vi "CSM - Run Script.vi"(0 "CSM Scripts":string, 1 "Current Module (\"\" to Generate an ID)":string, 7 "Continue If Error? (F)":bool, 9 "Wait (5000ms)":i32=5000, 11 "error in (no error)":errorcluster, 12 "Response Timeout (-2 Using Global Settings)":i32=-2) -> (4 "Response":string[](array[string]), 10 "Scripts Left":string, 15 "error out":errorcluster)   [LabVIEW 2017, in "Communicable State Machine.lvlib"]
doc: "Executes multiple CSM commands in a single batch, supporting synchronous messages, asynchronous messages, and registrations.\n\n<b>Temporary Variable Support</b>\n\nCSM - Run Script.vi supports an additional supplementary syntax to save return values to specified temporary variables for use in subsequent instructions. Use the `=>` symbol to save the return value to a variable, and variable names are case-insensitive. In subsequent instructions, you can reference the variable using the syntax `${variable name}`.\n\nExample:\n\n```\nAPI: Random -@ csm => var1\nAPI: Random -@ csm => var2\nAPI: echo >> ${var1} -@ csm\nAPI: echo >> ${var2} -@ csm\nAPI: echo >> ${var1},${var2} -@ csm\n```\n\n<b>Additional Command</b>\n\n- Wait: Wait for the specified number of milliseconds, for example `Wait: 1000` means wait 1000 milliseconds.\n\n```\nAPI: Do Something -@ csm\nWait: 1000 // Wait 1000 milliseconds, then continue to the next instruction\nAPI: Do Something Else -@ csm\n```\n\n> [!WARNING]\n> <b>Temporary Variable Support</b> and <b>Additional Command</b> are not natively supported by CSM, but are parsed and processed by CSM - Run Script.vi. Therefore, temporary variables can only be used within the same script execution and cannot be saved or passed across scripts. Wait is also not part of the CSM instructions and cannot use this syntax elsewhere.\n\n\n> [!NOTE] <b>CSM Message Target Module Description</b>\n>\n> In Normal Mode, the target module for a CSM message is the specified module name.\n> System-level modules start with a `.` in their name. The target module for a CSM message includes the `.` in the name. For example, if the requested module name is `.System`, the target module for the CSM message is `.System`.\n> In Worker Mode, the target module for a CSM message can only be the overall module name, not the node name. For example, if the requested module name is `Worker#`, the target module for the CSM message is `Worker`.\n> In Chain of Responsibility Mode, the target module for a CSM message can only be the overall module name, not the node name. For example, if the requested module name is `Chain$1`, the target module for the CSM message is `Chain`.\n\n\n-- <b>Controls</b> --\n- <b>Current Module (\"\" to Generate an ID)</b>: Name of the current module. If empty, a temporary ID is generated for debugging purposes to identify the location.\n- <b>CSM Scripts</b>: CSM commands to execute.\n- <b>Continue If Error? (F)</b>: Whether to continue execution if an error occurs. The default is FALSE, which specifies to not continue.\n- <b>Wait (5000 ms)</b>: Timeout duration for waiting module to be alive. The default is 5000 ms.\n- <b>Response Timeout (-2 Using Global Settings)</b>: Timeout for synchronous calls. The default is -2, which uses the global setting. You can set the global timeout using the CSM - Set TMO of Sync-Reply VI.\n\n-- <b>Indicators</b> --\n- <b>Response</b>: Returned results from executing the script. Only synchronous messages carry returns. The corresponding column for other commands will be an empty string.\n- <b>Scripts Left</b>: Remaining unexecuted scripts."
uses:
  Communicable State Machine.lvlib
  CSM - Broadcast Message Type.ctl
  _Shared/CSM Shared.lvlib
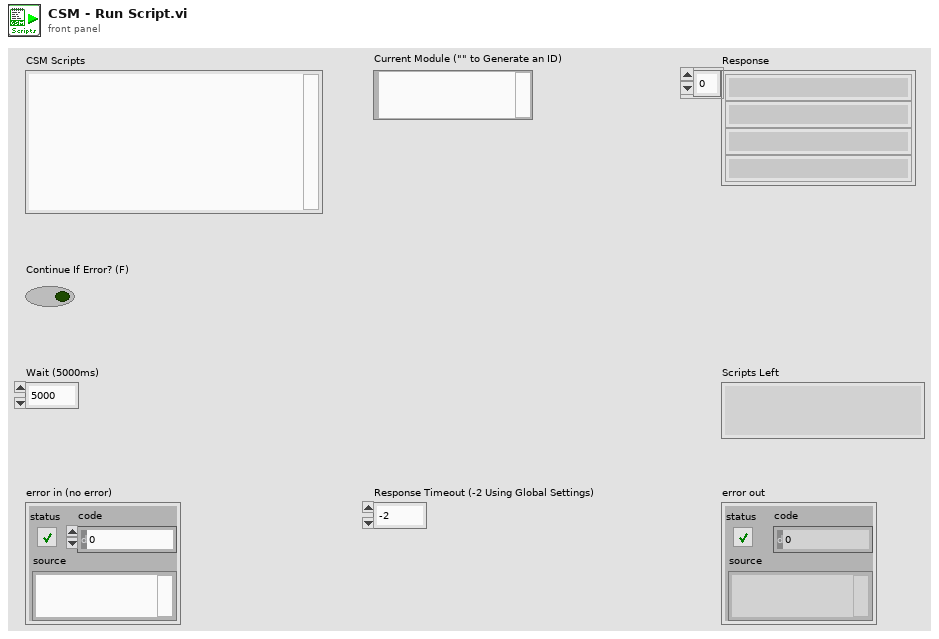
[diagram p1: front panel]
types:
  T1 = typedef "Communicable State Machine.lvlib/CSM - Broadcast Message Type.ctl" = enum16{"<Null>", "Status", "Interrupt"}
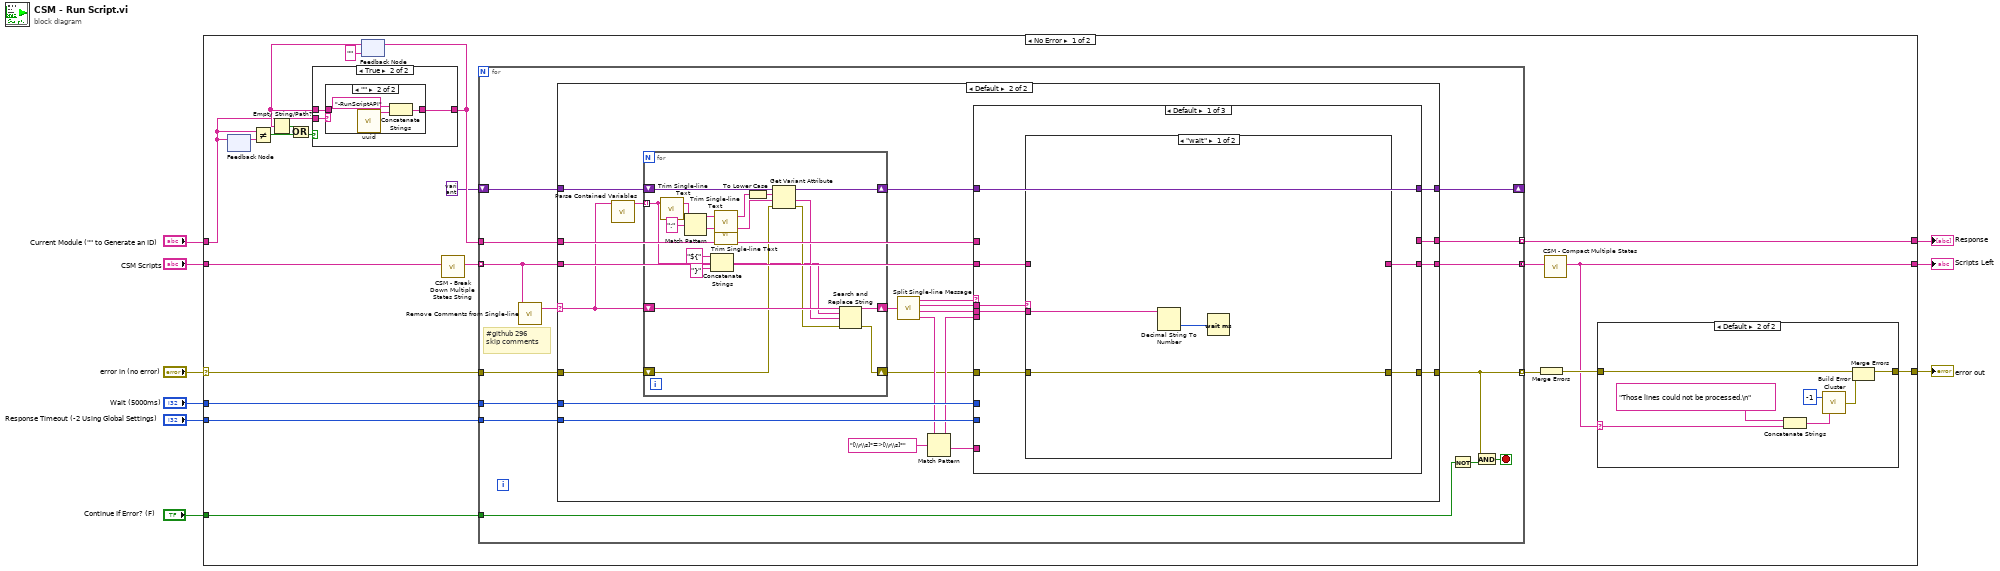
[diagram p0: block diagram]
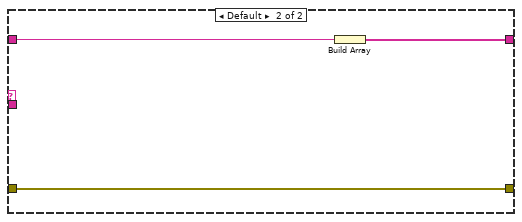
[diagram p6: hidden frame]
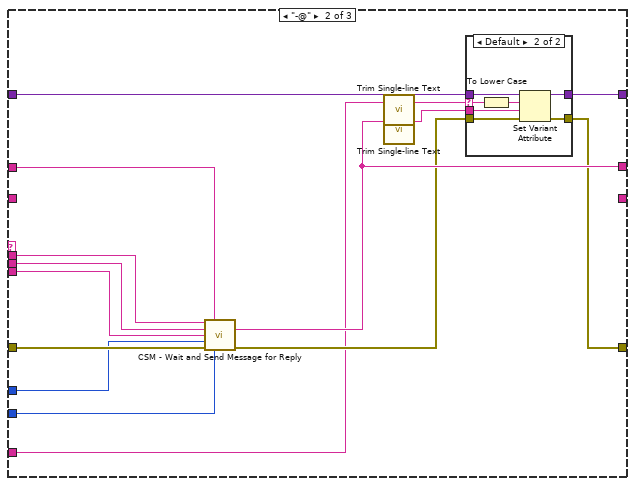
[diagram p7: hidden frame]
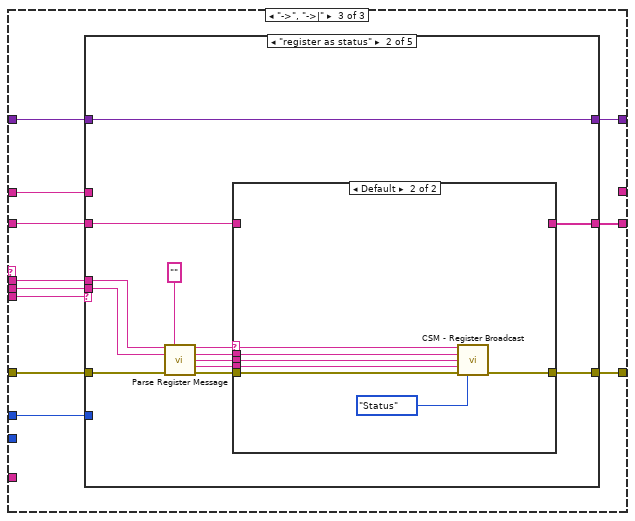
[diagram p9: hidden frame]
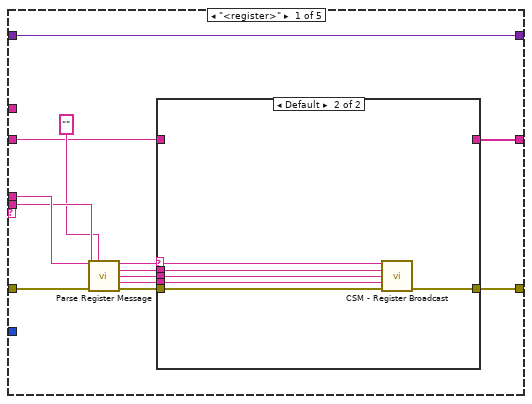
[diagram p10: hidden frame]
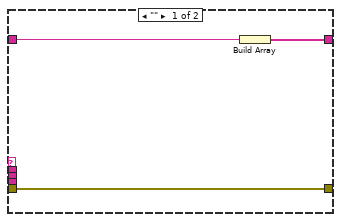
[diagram p11: hidden frame]
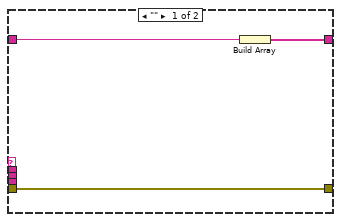
[diagram p12: hidden frame]
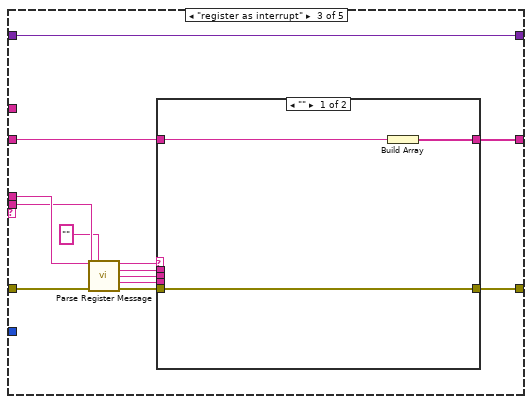
[diagram p13: hidden frame]
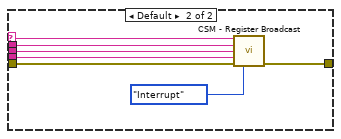
[diagram p14: hidden frame]
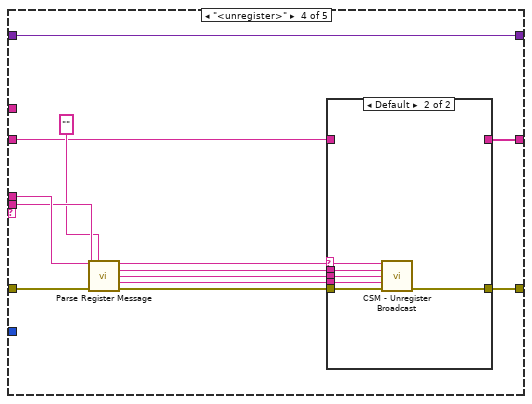
[diagram p15: hidden frame]
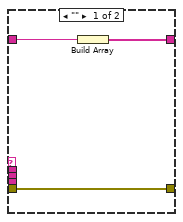
[diagram p16: hidden frame]
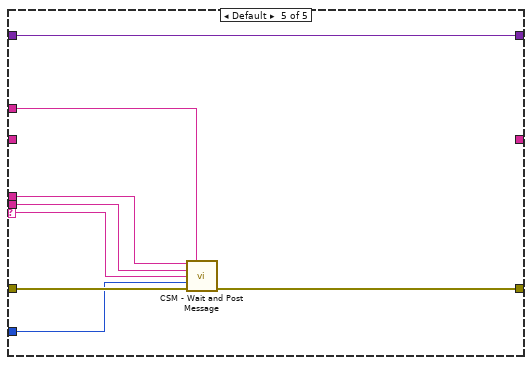
[diagram p17: hidden frame]
diagram:
  n1 = case shown="No Error" "error in (no error)" {
    selector: "error in (no error)" -> [w28 w246]
    tunnel: "CSM Scripts" -> [w27 _]
    tunnel: [w24 _] -> w7
    tunnel: [w23 w246] -> w6
    tunnel: "Current Module (\"\" to Generate an ID)" -> [w12 _]
    tunnel: "Response Timeout (-2 Using Global Settings)" -> [w22 _]
    tunnel: "Wait (5000ms)" -> [w21 _]
    tunnel: "Continue If Error? (F)" -> [w20 _]
    tunnel: [w19 _] -> w1
    frame No Error {
      n2 = feedback #1() -> (w18:string)  [unwired: 1 in]
      n3 = feedback-in #1(w12) -> ()
      n4 = Not Equal?(x=w12, y=w18) -> (x != y?=w17:bool)
      n5 = feedback #2("") -> (w14:string)
      n6 = Empty String/Path?(string/path=w14) -> (empty?=w13:bool)
      n7 = Or(x=w13, y=w17) -> (x .or. y?=w15:bool)
      n8 = case shown="True" w15 {
        tunnel: w14 -> [w31 w34]
        tunnel: w12 -> [_ w33]
        tunnel: [w31 w32] -> w11
        frame False {
        }
        frame True {
          n9 = case shown="\"\"" w33 {
            selector: w33 -> [w35 _]
            tunnel: [w35 w36] -> w32
            tunnel: w34 -> [_ _]
            frame Default {
            }
            frame "" {
              n10 = call "uuid.vi"() -> ("UUID"=w37:string)  [unwired: 11 in]
              n11 = Concatenate Strings("-RunScriptAPI" ("Name (\"\" to Use UUID)"), w37) -> (w36:string)
            }
          }
        }
      }
      n12 = feedback-in #2(w11) -> ()
      n13 = call "CSM - Break Down Multiple States String.vi"("States"=w27) -> ("Multiple States"=w26:string[])  [unwired: 10 in]
      n14 = for {
        tunnel: w26 -> [w57] mode=indexing
        tunnel: w28 -> [w60]
        tunnel: [w52] -> w29 mode=indexing
        tunnel: [w58] -> w25 mode=concatenating
        tunnel: w11 -> [w56]
        tunnel: w22 -> [w55]
        tunnel: w21 -> [w54]
        tunnel: w20 -> [w51]
        tunnel: [w49] -> w19 mode=indexing
        shift-right: [w48] -> _
        shift-left: variant -> [w47]
        stop <- w53 stop-if-true
        # "#github 296\nskip comments"
        n15 = call "Remove Comments from Single-line.vi"("single-line text"=w57) -> ("single-line text without comments"=w59:string)  [unwired: 2 in]
        n16 = case shown="Default" w59 {
          selector: w59 -> [_ w65]
          tunnel: [w62 w84] -> w52
          tunnel: w60 -> [w62 w64]
          tunnel: [_ w80] -> w58
          tunnel: w57 -> [_ w79]
          tunnel: w56 -> [_ w78]
          tunnel: w55 -> [_ w77]
          tunnel: w54 -> [_ w76]
          tunnel: [_ w75] -> w49
          tunnel: [w61 w74] -> w48
          tunnel: w47 -> [w61 w69]
          frame "" {
          }
          frame Default {
            n17 = call "Parse Contained Variables.vi"("String"=w65) -> ("Contained Variables"=w67:string[])  [unwired: 9 in, 1 out]
            n18 = for {
              shift-right: [w101] -> w68
              shift-left: w69 -> [w103]
              tunnel: w67 -> [w88] mode=indexing
              shift-right: [w94] -> w66
              shift-left: w65 -> [w93]
              shift-right: [w91] -> w63
              shift-left: w64 -> [w92]
              n19 = call "Trim Single-line Text.vi"("single-line text"=w88) -> ("trimed text"=w98:string)  [unwired: 2 in]
              n20 = Match Pattern(string=w98, regular expression=":") -> (before substring=w100:string, after substring=w99:string)  [unwired: 1 in, 2 out]
              n21 = Concatenate Strings("${" ("regular expression"), w88, "}" ("regular expression")) -> (w85:string)
              n22 = call "Trim Single-line Text.vi"("single-line text"=w100) -> ("trimed text"=w97:string)  [unwired: 2 in]
              n23 = call "Trim Single-line Text.vi"("single-line text"=w99) -> ("trimed text"=w96:string)  [unwired: 2 in]
              n24 = To Lower Case(string=w97) -> (all lower case string=w95:string)
              n25 = Get Variant Attribute(Variant=w103, name=w95, default value (empty Variant)=w96, error in=w92) -> (duplicate Variant=w101:variant, value=w89:string, error out=w90:errorcluster)  [unwired: 1 out]
              n26 = Search and Replace String(input string=w93, search string=w85, replace string=w89, error in=w90) -> (result string=w94:string, error out=w91:errorcluster)  [unwired: 4 in, 2 out]
            }
            n27 = call "Split Single-line Message.vi"("single-line text"=w66) -> ("operator"=w83:string, "state"=w81:string, "args"=w82:string, "source/target"=w72:string)  [unwired: 6 in]
            n28 = Match Pattern(string=w72, regular expression="[\\r\\s]*=>[\\r\\s]*") -> (before substring=w71:string, after substring=w70:string)  [unwired: 1 in, 2 out]
            n29 = case shown="Default" w83 {
              tunnel: w71 -> [_ w131 w151]
              tunnel: w82 -> [w104 w130 w150]
              tunnel: w81 -> [w105 w129 w149]
              tunnel: w63 -> [w106 w128 w148]
              tunnel: [w107 w120 w147] -> w84
              tunnel: [w110 _ w146] -> w80
              tunnel: w79 -> [w109 _ w145]
              tunnel: w78 -> [_ w127 w144]
              tunnel: w77 -> [_ w126 _]
              tunnel: w76 -> [_ w125 w143]
              tunnel: [_ w122 _] -> w75
              tunnel: [w108 w123 w142] -> w74
              tunnel: w68 -> [w108 w124 w141]
              tunnel: w70 -> [_ w119 _]
              frame Default {
                n30 = case shown="\"wait\"" w105 {
                  tunnel: [_ w116] -> w110
                  tunnel: w109 -> [_ w115]
                  tunnel: [w113 w114] -> w107
                  tunnel: w106 -> [w113 w114]
                  tunnel: w104 -> [w112 _]
                  frame "wait" {
                    n31 = Decimal String To Number(string=w112) -> (number=w111:i32)  [unwired: 2 in, 1 out]
                    n32 = Wait (ms)(milliseconds to wait=w111) -> ()  [unwired: 1 out]
                  }
                  frame Default {
                    n33 = Build Array(w115) -> (w116:string[])
                  }
                }
              }
              frame "-@" {
                n34 = call "CSM - Wait and Send Message for Reply.vi"("State"=w129, "Current Module (\"\" to Generate an ID)"=w127, "Arguments (\"\")"=w130, "Target Module"=w131, "Wait (5000ms)"=w125, "Error In (No Error)"=w128, "Response Timeout (-2 Using Global Settings)"=w126) -> ("Response"=w122:string, "error out"=w121:errorcluster)  [unwired: 5 in, 2 out]
                n35 = call "Trim Single-line Text.vi"("single-line text"=w119) -> ("trimed text"=w118:string)  [unwired: 2 in]
                n36 = call "Trim Single-line Text.vi"("single-line text"=w122) -> ("trimed text"=w117:string)  [unwired: 2 in]
                n37 = case shown="Default" w118 {
                  selector: w118 -> [_ w136]
                  tunnel: w124 -> [w133 w140]
                  tunnel: [w133 w139] -> w123
                  tunnel: w121 -> [w132 w138]
                  tunnel: [w132 w137] -> w120
                  tunnel: w117 -> [_ w135]
                  frame "" {
                  }
                  frame Default {
                    n38 = To Lower Case(string=w136) -> (all lower case string=w134:string)
                    n39 = Set Variant Attribute(Variant=w140, name=w134, value=w135, error in=w138) -> (Variant out=w139:variant, error out=w137:errorcluster)  [unwired: 1 out]
                  }
                }
              }
              frame "->", "->|" {
                n40 = case shown="\"register as status\"" w151 {
                  selector: w151 -> [_ _ _ _ w245]
                  tunnel: w150 -> [w158 w179 w201 w223 w244]
                  tunnel: w149 -> [w159 w180 w202 w224 w243]
                  tunnel: w148 -> [w157 w178 w200 w222 w242]
                  tunnel: [w156 w177 w199 w221 w241] -> w147
                  tunnel: [w154 w175 w197 w219 _] -> w146
                  tunnel: w145 -> [w153 w174 w196 w218 _]
                  tunnel: w144 -> [_ _ _ _ w240]
                  tunnel: w143 -> [_ _ _ _ w239]
                  tunnel: [w152 w173 w195 w217 w238] -> w142
                  tunnel: w141 -> [w152 w173 w195 w217 w238]
                  frame "<register>" {
                    n41 = call "Parse Register Message.vi"("State"=w159, "Module Name"="", "Args"=w158) -> ("Target"=w163:string, "Source"=w162:string, "Status"=w161:string, "Api"=w160:string)  [unwired: 8 in, 1 out]
                    n42 = case shown="Default" w163 {
                      selector: w163 -> [_ w172]
                      tunnel: w162 -> [_ w171]
                      tunnel: w161 -> [_ w170]
                      tunnel: w160 -> [_ w169]
                      tunnel: w157 -> [w166 w168]
                      tunnel: [w166 w167] -> w156
                      tunnel: [w164 _] -> w154
                      tunnel: w153 -> [w165 _]
                      frame "" {
                        n43 = Build Array(w165) -> (w164:string[])
                      }
                      frame Default {
                        n44 = call "CSM - Register Broadcast.vi"("CSM Name(Empty for Broadcast Event)"=w172, "Source CSM Name (* as Default)"=w171, "Trigger"=w170, "API (If \"\", Same as Trigger)"=w169, "Error In"=w168) -> ("error out"=w167:errorcluster)  [unwired: 9 in, 1 out]
                      }
                    }
                  }
                  frame "register as status" {
                    n45 = call "Parse Register Message.vi"("State"=w180, "Module Name"="", "Args"=w179) -> ("Target"=w184:string, "Source"=w183:string, "Status"=w182:string, "Api"=w181:string)  [unwired: 8 in, 1 out]
                    n46 = case shown="Default" w184 {
                      selector: w184 -> [_ w194]
                      tunnel: w183 -> [_ w193]
                      tunnel: w182 -> [_ w192]
                      tunnel: w181 -> [_ w191]
                      tunnel: w178 -> [w187 w190]
                      tunnel: [w187 w189] -> w177
                      tunnel: [w185 _] -> w175
                      tunnel: w174 -> [w186 _]
                      frame "" {
                        n47 = Build Array(w186) -> (w185:string[])
                      }
                      frame Default {
                        n48 = call "CSM - Register Broadcast.vi"("CSM Name(Empty for Broadcast Event)"=w194, "Source CSM Name (* as Default)"=w193, "Trigger"=w192, "API (If \"\", Same as Trigger)"=w191, "Error In"=w190, "Priority (No Change)"=CSM_-_Broadcast_Message_Type."Status") -> ("error out"=w189:errorcluster)  [unwired: 8 in, 1 out]
                      }
                    }
                  }
                  frame "register as interrupt" {
                    n49 = call "Parse Register Message.vi"("State"=w202, "Module Name"="", "Args"=w201) -> ("Target"=w206:string, "Source"=w205:string, "Status"=w204:string, "Api"=w203:string)  [unwired: 8 in, 1 out]
                    n50 = case shown="\"\"" w206 {
                      selector: w206 -> [_ w216]
                      tunnel: w205 -> [_ w215]
                      tunnel: w204 -> [_ w214]
                      tunnel: w203 -> [_ w213]
                      tunnel: w200 -> [w209 w212]
                      tunnel: [w209 w211] -> w199
                      tunnel: [w207 _] -> w197
                      tunnel: w196 -> [w208 _]
                      frame "" {
                        n51 = Build Array(w208) -> (w207:string[])
                      }
                      frame Default {
                        n52 = call "CSM - Register Broadcast.vi"("CSM Name(Empty for Broadcast Event)"=w216, "Source CSM Name (* as Default)"=w215, "Trigger"=w214, "API (If \"\", Same as Trigger)"=w213, "Error In"=w212, "Priority (No Change)"=CSM_-_Broadcast_Message_Type."Interrupt") -> ("error out"=w211:errorcluster)  [unwired: 8 in, 1 out]
                      }
                    }
                  }
                  frame "<unregister>" {
                    n53 = call "Parse Register Message.vi"("State"=w224, "Module Name"="", "Args"=w223) -> ("Target"=w228:string, "Source"=w227:string, "Status"=w226:string, "Api"=w225:string)  [unwired: 8 in, 1 out]
                    n54 = case shown="Default" w228 {
                      selector: w228 -> [_ w237]
                      tunnel: w227 -> [_ w236]
                      tunnel: w226 -> [_ w235]
                      tunnel: w225 -> [_ w234]
                      tunnel: w222 -> [w231 w233]
                      tunnel: [w231 w232] -> w221
                      tunnel: [w229 _] -> w219
                      tunnel: w218 -> [w230 _]
                      frame "" {
                        n55 = Build Array(w230) -> (w229:string[])
                      }
                      frame Default {
                        n56 = call "CSM - Unregister Broadcast.vi"("CSM Name(Empty for Broadcast Event)"=w237, "Source CSM Name (* as Default)"=w236, "Trigger"=w235, "API (\"*\" as Default)"=w234, "Error In"=w233) -> ("error out"=w232:errorcluster)  [unwired: 9 in, 1 out]
                      }
                    }
                  }
                  frame Default {
                    n57 = call "CSM - Wait and Post Message.vi"("State"=w243, "Current Module (\"\" to Generate an ID)"=w240, "Arguments (\"\")"=w244, "Target Module"=w245, "Wait (5000ms)"=w239, "Error In (No Error)"=w242) -> ("error out"=w241:errorcluster)  [unwired: 8 in, 1 out]
                  }
                }
              }
            }
          }
        }
        n58 = Not(x=w51) -> (.not. x?=w50:bool)
        n59 = And(x=w52, y=w50) -> (x .and. y?=w53:bool)
      }
      n60 = Merge Errors(w29) -> (w30:errorcluster)
      n61 = call "CSM - Compact Multiple States.vi"("Multiple States"=w25) -> ("States"=w24:string)  [unwired: 9 in]
      n62 = case shown="Default" w24 {
        selector: w24 -> [_ w42]
        tunnel: w30 -> [w39 w46]
        tunnel: [w39 w41] -> w23
        frame "" {
        }
        frame Default {
          n63 = Concatenate Strings("Those lines could not be processed.\n" ("String to Prepend to source (\"\")"), w42) -> (w43:string)
          n64 = call "Build Error Cluster.vi"("String to Prepend to Source (\"\")"=w43, "Code"=-1 ("code")) -> ("error out"=w40:errorcluster)
          n65 = Merge Errors(w46, w40) -> (w41:errorcluster)
        }
      }
    }
    frame Error {
    }
  }
  "error out" <- w6
  "Scripts Left" <- w7
  "Response" <- w1
